vi "ReadAIs.vi"(7 "GroveConnector":enum16{"A0", "A1", "A2"}(ring), 8 "error in (no error)":errorcluster, 11 "Session in":refnum<class "Session.lvclass">) -> (0 "error out":errorcluster, 2 "Value":T1, 3 "Session out":refnum<class "Session.lvclass">)   [LabVIEW 2020]
uses:
  CTI/Raw ADC.ctl
  CTI/Session/Session.lvclass
  CTI/ADC Number.ctl
  CTI/CTI.lvlib
panel:
  # "Input"
  # "Output"
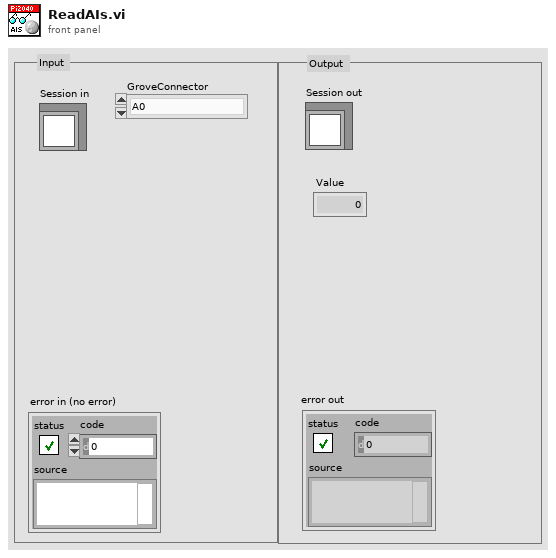
[diagram p1: front panel]
types:
  T1 = typedef "CTI.lvlib/Raw ADC.ctl" = u16
  T2 = typedef "CTI.lvlib/ADC Number.ctl" = i8
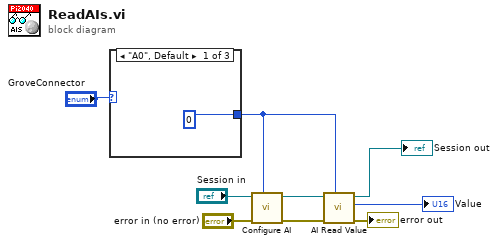
[diagram p0: block diagram]
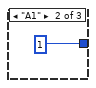
[diagram p2: hidden frame]
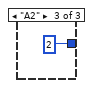
[diagram p3: hidden frame]
diagram:
  n1 = case shown="\"A0\", Default" "GroveConnector" {
    tunnel: [T2 0 T2 1 T2 2] -> w6
    frame "A0", Default {
    }
    frame "A1" {
    }
    frame "A2" {
    }
  }
  n2 = call "Configure AI.vi"("ADC #"=w6, "error in (no error)"="error in (no error)", "Session in"="Session in") -> ("error out"=w9:errorcluster, "Session out"=w8:refnum<class "Session.lvclass">)  [unwired: 7 in]
  n3 = call "AI Read Value.vi"("ADC #"=w6, "error in (no error)"=w9, "Session in"=w8) -> ("error out"=→"error out":errorcluster, "Value"=→"Value":T1, "Session out"=→"Session out":refnum<class "Session.lvclass">)  [unwired: 6 in]
